vi "Registry Logging.vi"() -> ()   [LabVIEW 2018]
uses:
  src/api/logger_class/Log Levels.ctl
  ff44e4a9-c346-414c-ae2a-efcf3ff82913.vi
  593378fc-b3d1-4ba2-990a-aac09aa27d13.vi
  cbe71786-2e87-4bc7-85be-dae61289713f.vi
  c9322c4e-9f12-43bd-adb9-b3674d2f7074.vi
  593378fc-b3d1-4ba2-990a-aac09aa27d13.vi/6f202c45-f0ca-42f4-9f63-a87d9fe0c32d.vi
  src/api/Log.vi
  cbe71786-2e87-4bc7-85be-dae61289713f.vi/73f0ec31-6bdf-4568-9d3b-fef50ac01b30.vi
  c9322c4e-9f12-43bd-adb9-b3674d2f7074.vi/0a1ee2ab-da6d-4243-8cf3-8125e611a602.vi
  src/api/configuration/filters/regex_filter/Regex.lvclass
  C:/Users/Colin/Documents/software_projects/labview/glog/src/api/extension/filter_interface/Filter.lvclass
  src/api/configuration/scopes/basic_scope/Basic.lvclass
  C:/Users/Colin/Documents/software_projects/labview/glog/src/api/extension/scope_interface/Scope.lvclass
  src/api/configuration/formatters/format_string_formatter/Format String.lvclass
  C:/Users/Colin/Documents/software_projects/labview/glog/src/api/extension/formatter_interface/Formatter.lvclass
  src/api/configuration/handlers/file_handler/File Handler.lvclass
  C:/Users/Colin/Documents/software_projects/labview/glog/src/api/extension/formatting_handler_interface/Formatting Handler.lvclass
  src/api/configuration/filters/regex_filter/New (Element).vi
  src/api/configuration/scopes/basic_scope/New (Element).vi
  src/registry/Log.vi
  src/api/logger_class/Logger.lvclass
  src/api/GLog.lvlib
panel:
  out "ms timer":u32[](array[numeric])
  out "elapsed time":u32[](array[numeric])
  out "iterations":i32[](array[numeric])
  in  "error in (no error)":errorcluster
  out "error out":errorcluster
  in  "total iterations":i32=30
  # "Locals"
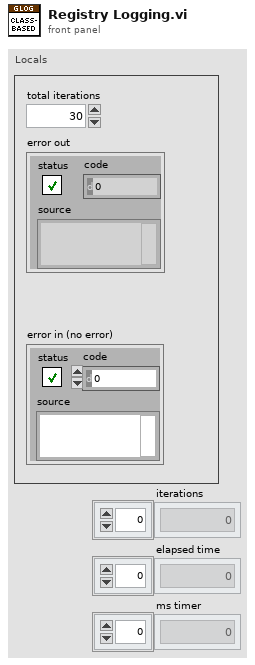
[diagram p1: front panel]
types:
  T1 = typedef "GLog.lvlib/Logger.lvclass/Log Levels.ctl" = enum16{"Trace", "Debug", "Info", "Warning", "Error", "Critical"}
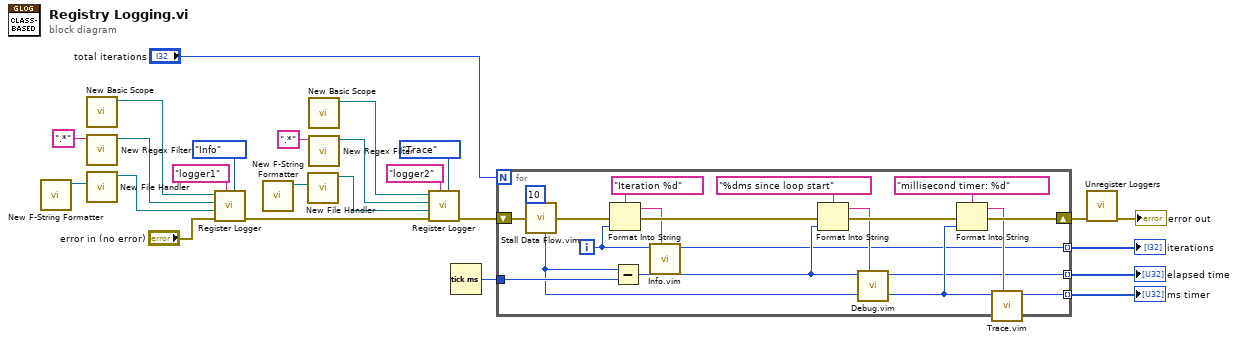
[diagram p0: block diagram]
diagram:
  n1 = call "New F-String Formatter.vi"() -> ("new f-string formatter"=w12:refnum<class "Format String.lvclass">)  [unwired: 11 in]
  n2 = call-poly "New Basic Scope.vi"() -> ("basic scope"=w15:refnum<class "Basic.lvclass">)  [unwired: 11 in]
  n3 = call-poly "New Regex Filter.vi"("regex string"=".*") -> ("regex out"=w14:refnum<class "Regex.lvclass">)  [unwired: 9 in, 1 out]
  n4 = call "New File Handler.vi"("formatter (JSON)"=w12) -> ("file handler"=w13:refnum<class "File Handler.lvclass">)  [unwired: 8 in, 2 out]
  n5 = call "Register Logger.vi"("minimum log level (Info)"=Log_Levels."Info" ("minimum log level"), "name (\"Default\")"="logger1" ("name (\"Default\")"), "error in (no error)"="error in (no error)", "log handler (file handler)"=w13, "log filter (none)"=w14, "logger scope (all)"=w15) -> ("error out"=w3:errorcluster)  [unwired: 5 in]
  n6 = call "New F-String Formatter.vi"() -> ("new f-string formatter"=w7:refnum<class "Format String.lvclass">)  [unwired: 11 in]
  n7 = call "New File Handler.vi"("formatter (JSON)"=w7) -> ("file handler"=w8:refnum<class "File Handler.lvclass">)  [unwired: 8 in, 2 out]
  n8 = call-poly "New Basic Scope.vi"() -> ("basic scope"=w10:refnum<class "Basic.lvclass">)  [unwired: 11 in]
  n9 = call-poly "New Regex Filter.vi"("regex string"=".*") -> ("regex out"=w9:refnum<class "Regex.lvclass">)  [unwired: 9 in, 1 out]
  n10 = call "Register Logger.vi"("minimum log level (Info)"=Log_Levels."Trace" ("minimum log level"), "name (\"Default\")"="logger2" ("name (\"Default\")"), "error in (no error)"=w3, "log handler (file handler)"=w8, "log filter (none)"=w9, "logger scope (all)"=w10) -> ("error out"=w4:errorcluster)  [unwired: 5 in]
  n11 = Tick Count (ms)() -> (millisecond timer value=w24:u32)
  n12 = for {
    N: "total iterations" -> [_]
    tunnel: w24 -> [w43]
    shift-right: [w36] -> w22
    shift-left: w4 -> [w29]
    tunnel: [w27] -> w20 mode=indexing
    tunnel: [w26] -> w19 mode=indexing
    tunnel: [w25] -> w18 mode=indexing
    i -> [w35]
    n13 = call "Stall Data Flow.vim"("value in"=w29, "milliseconds to wait"=u32 10 ("loop iteration delay [ms]")) -> ("millisecond timer value"=w31:u32, "value out"=w28:errorcluster)
    n14 = Format Into String(format string="Iteration %d" ("message"), error in=w28, w35) -> (resulting string=w34:string, error out=w38:errorcluster)  [unwired: 1 in]
    n15 = Subtract(x=w31, y=w43) -> (x-y=w32:u32)
    n16 = call "Info.vim"("data in (null)"=w35, "message"=w34) -> ("data out"=w27:i32)  [unwired: 9 in]
    n17 = Format Into String(format string="%dms since loop start" ("message"), error in=w38, w32) -> (resulting string=w33:string, error out=w37:errorcluster)  [unwired: 1 in]
    n18 = call "Debug.vim"("data in (null)"=w32, "message"=w33) -> ("data out"=w26:u32)  [unwired: 9 in]
    n19 = Format Into String(format string="millisecond timer: %d" ("message"), error in=w37, w31) -> (resulting string=w30:string, error out=w36:errorcluster)  [unwired: 1 in]
    n20 = call "Trace.vim"("data in (null)"=w31, "message"=w30) -> ("data out"=w25:u32)  [unwired: 9 in]
  }
  "iterations" <- w20
  "elapsed time" <- w19
  "ms timer" <- w18
  n21 = call "Unregister Loggers.vi"("error in (no error)"=w22) -> ("error out"=→"error out":errorcluster)  [unwired: 9 in, 1 out]
